vi "RDV-addDataToDupMapFromFile.vi"(7 "Folder Path":path=path "C:/projects/Universitet/Master/data/Real Test - First libreVNA test with calibration file/Converted Data", 8 "error in (no error)":errorcluster, 11 "RDV-Reflection_Data_viewer in":refnum<class "RDV-Reflection_Data_viewer.lvclass">) -> (0 "error out":errorcluster, 2 "Keys":string[](array[string]), 3 "RDV-Reflection_Data_viewer out":refnum<class "RDV-Reflection_Data_viewer.lvclass">)   [LabVIEW 2020, in "RDV-Reflection_Data_viewer.lvclass"]
doc: "Reads every common-format file in a folder and adds the data to the viewer's map, numbering the keys. Returns the keys."
uses:
  RDV-Reflection_Data_viewer.lvclass
  Computation/RDC-perm_calc_type.ctl
  Reflector/RFH-Reflection_File_Handler.lvlib
  Computation/RDC-Reflection_Data_Computation.lvlib
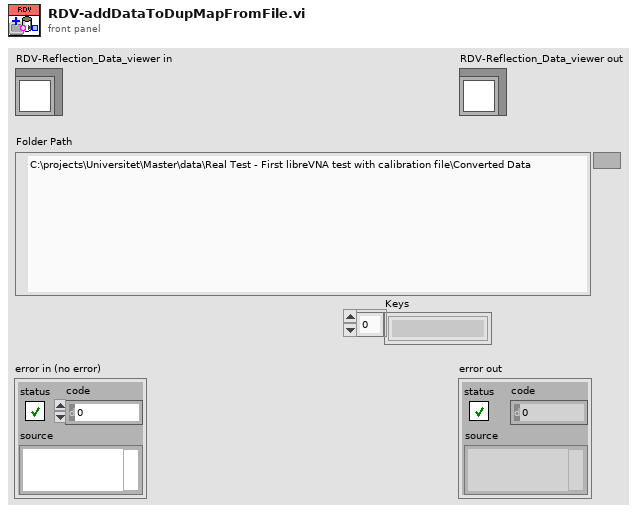
[diagram p1: front panel]
types:
  T1 = typedef "RDC-Reflection_Data_Computation.lvlib/RDC-perm_calc_type.ctl" = enum16{"Basic", "Capacative", "Advance", "Bilinear", "Size"}
  T2 = typedef "RFH-Reflection_File_Handler.lvlib/RFH-common_data_format.ctl" = cluster{"Frequency":dbl[], "Reflection'":dbl[], "Reflection''":dbl[], "Permativity'":dbl[], "Permativity''":dbl[], "Conductivity":dbl[], "Loss Tangent":dbl[], "Resistance":dbl[], "Reactance":dbl[]}
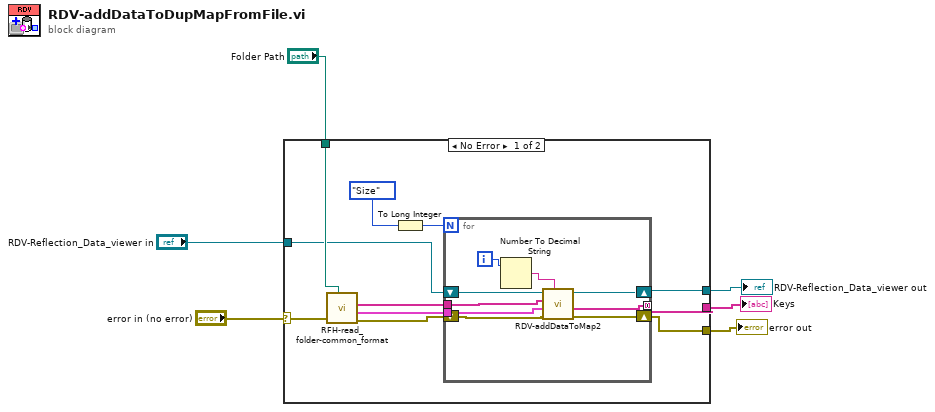
[diagram p0: block diagram]
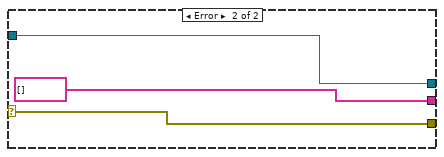
[diagram p2: hidden frame]
diagram:
  n1 = case shown="No Error" "error in (no error)" {
    selector: "error in (no error)" -> [w16 w29]
    tunnel: [w10 w29] -> w5
    tunnel: [w13 w28] -> w3
    tunnel: "RDV-Reflection_Data_viewer in" -> [w15 w28]
    tunnel: "Folder Path" -> [w17 _]
    tunnel: [w12 string[] []] -> w1
    frame No Error {
      n2 = call "RFH-read_folder-common_format.vi"("File Path"=w17, "error In"=w16) -> ("error out"=w11:errorcluster, "Data"=w14:T2[], "Names"=w7:string[])  [unwired: 7 in]
      n3 = To Long Integer(number=RDC-perm_calc_type."Size" ("Perm calc type")) -> (32bit integer=w8:i32)
      n4 = for {
        N: w8 -> [_]
        tunnel: w7 -> [w18]
        tunnel: w14 -> [w21]
        tunnel: [w24] -> w12 mode=concatenating
        shift-right: [w23] -> w13
        shift-left: w15 -> [w22]
        shift-right: [w25] -> w10
        shift-left: w11 -> [w26]
        i -> [w20]
        n5 = Number To Decimal String(number=w20) -> (decimal integer string=w19:string)  [unwired: 1 in]
        n6 = call "RDV-addDataToMap2.vi"("Add mod"=w19, "error in (no error)"=w26, "Data"=w21, "Names"=w18, "RDV-Reflection_Data_viewer in"=w22) -> ("error out"=w25:errorcluster, "Keys"=w24:string[], "RDV-Reflection_Data_viewer out"=w23:refnum<class "RDV-Reflection_Data_viewer.lvclass">)  [unwired: 4 in]
      }
    }
    frame Error {
    }
  }
  "error out" <- w5
  "RDV-Reflection_Data_viewer out" <- w3
  "Keys" <- w1
